vi "Get Module Direction.vi"(8 "error in (no error)":errorcluster, 11 "Module in":refnum<class "Module.lvclass">) -> (0 "error out":errorcluster, 2 "Direction":enum16{"Input", "Output"}(ring), 3 "Module out":refnum<class "Module.lvclass">)   [LabVIEW 2019, in "Module.lvclass"]
uses:
  Module.lvclass
  Module Configuration.ctl
  Module.lvclass/Module.ctl
  VI/Module Loop/Module Loop.lvclass
  <vilib>/Utility/Data Type/NI_Data Type.lvlib
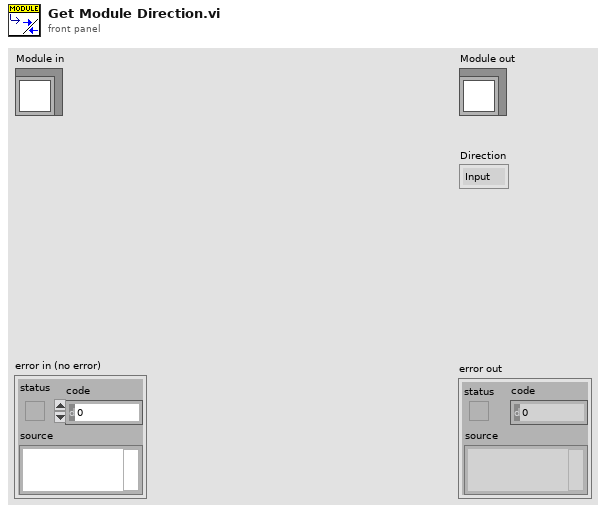
[diagram p1: front panel]
types:
  T1 = typedef "Module Loop.lvclass/Module Configuration.ctl" = cluster{"Type":string, "Direction":string, "Speed":string, "Channels":string, "FXP Type":string}
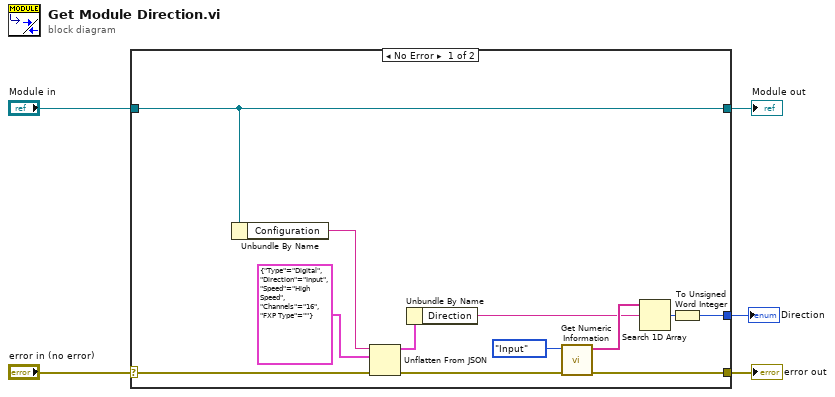
[diagram p0: block diagram]
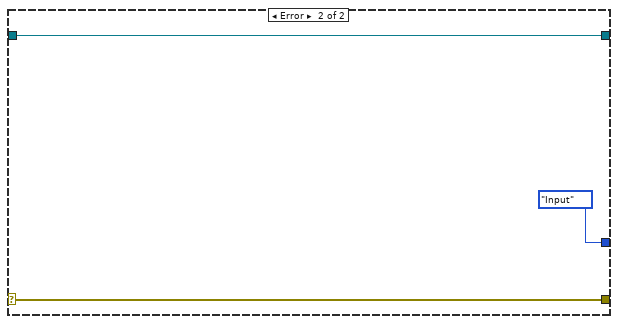
[diagram p2: hidden frame]
diagram:
  n1 = case shown="No Error" "error in (no error)" {
    selector: "error in (no error)" -> [w15 w20]
    tunnel: [w6 w20] -> w4
    tunnel: [w17 w19] -> w2
    tunnel: "Module in" -> [w17 w19]
    tunnel: [w8 enum16{"Input", "Output"}."Input" ("Direction")] -> w1
    frame No Error {
      n2 = Unbundle By Name(w17) -> ("Configuration"=w16:string)
      n3 = Unflatten From JSON(JSON string=w16, type and defaults=T1 {"Type"="Digital", "Direction"="Input", "Speed"="High Speed", "Channels"="16", "FXP Type"=""} ("Cluster"), error in (no error)=w15) -> (value=w13:T1, error out=w7:errorcluster)  [unwired: 4 in]
      n4 = Unbundle By Name(w13) -> ("Direction"=w10:string)
      n5 = call <vilib>:"Get Numeric Information.vi"("error in (no error)"=w7, "variant"=enum16{"Input", "Output"}."Input" ("Direction")) -> ("error out"=w6:errorcluster, "enum names"=w11:string[])  [unwired: 6 in, 2 out]
      n6 = Search 1D Array(1D array=w11, element=w10) -> (index of element=w9:i32)  [unwired: 1 in]
      n7 = To Unsigned Word Integer(number=w9) -> (unsigned 16bit integer=w8:u16)
    }
    frame Error {
    }
  }
  "error out" <- w4
  "Module out" <- w2
  "Direction" <- w1
